vi "Time profile graph.vi"(8 "Assigned Time Profile plus":T1, 10 "time":dbl[](array[numeric]), 11 "Relative Data Array":dbl[](array[numeric])) -> (3 "Signal Time Graph":cluster{"time":dbl[], "current":dbl[]}[](graph))   [LabVIEW 2018]
panel:
  in  "Assigned Time Profile":T2
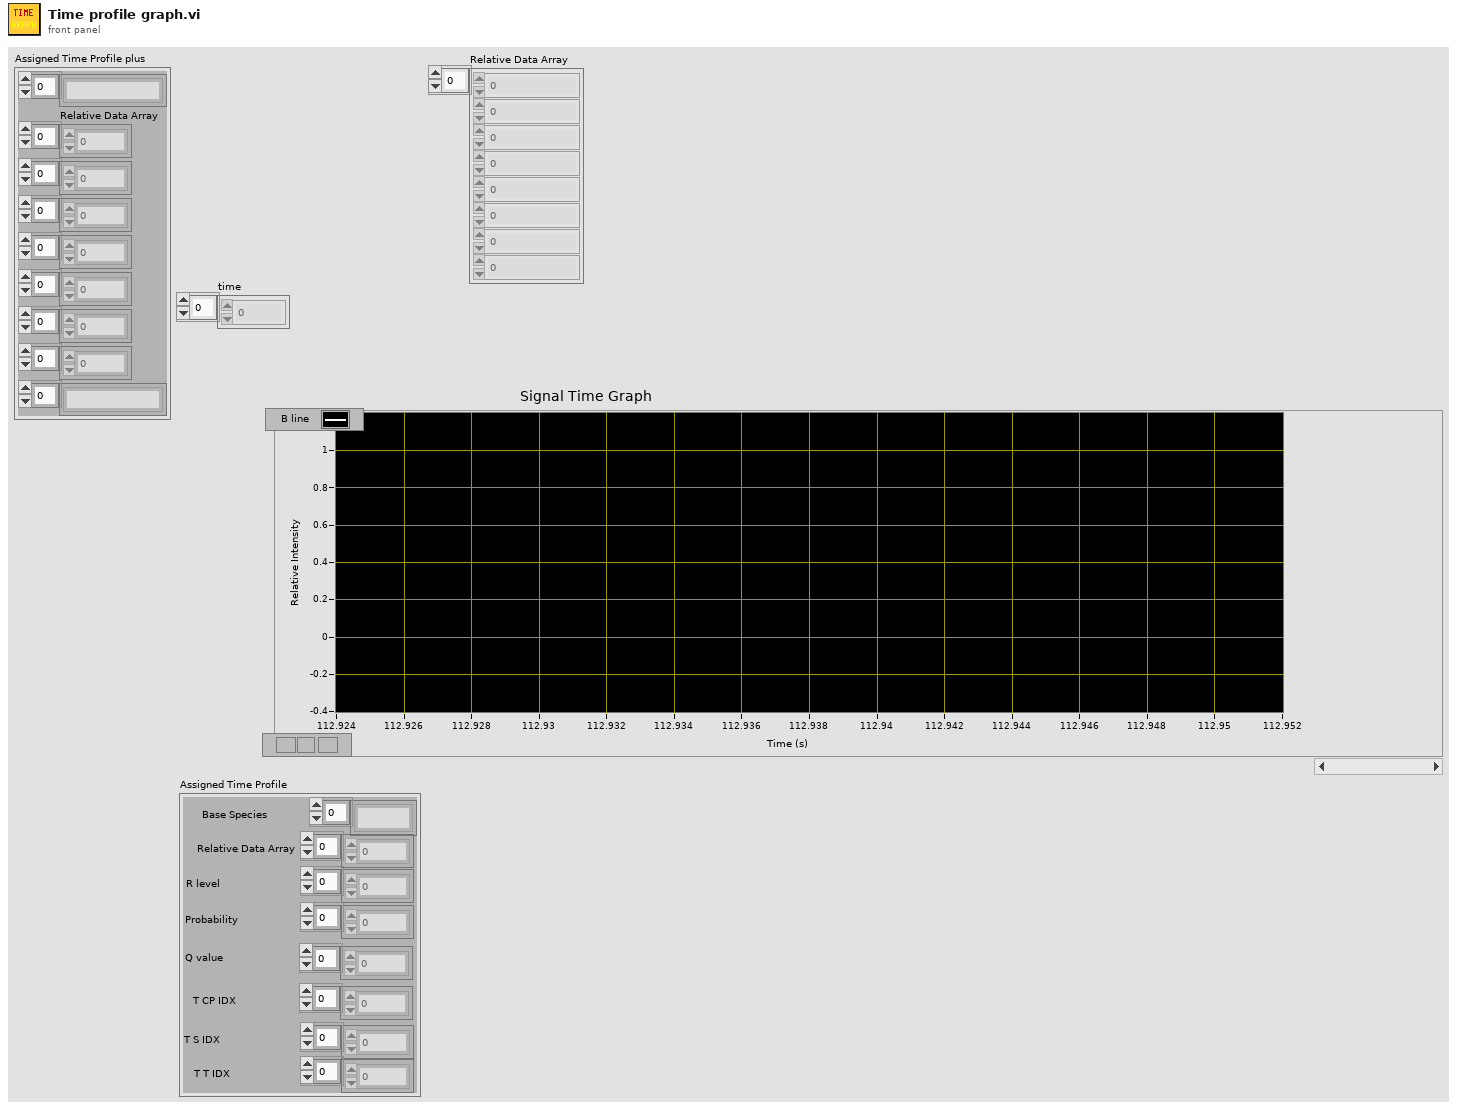
[diagram p1: front panel]
types:
  T1 = cluster{string[], "Relative Data Array":dbl[], dbl[], dbl[], dbl[], i32[], i32[], i32[], string[]}
  T2 = cluster{"Base Species":string[], "Relative Data Array":dbl[], "R level":dbl[], "Probability":dbl[], "Q value":dbl[], "T CP IDX":i32[], "T S IDX":i32[], "T T IDX":i32[]}
  T3 = cluster{"time":dbl[], "Relative Data Array":dbl[]}
  T4 = cluster{"time":dbl[], "Relative Data Array":dbl[]}[]
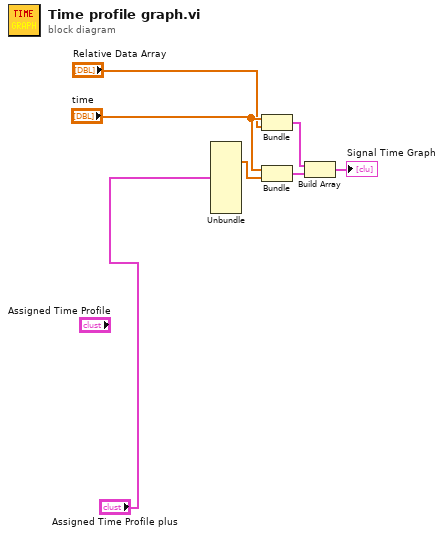
[diagram p0: block diagram]
diagram:
  n1 = Unbundle("Assigned Time Profile plus") -> (w2:dbl[])  [unwired: 8 out]
  n2 = Bundle("time"="time", "Relative Data Array"="Relative Data Array") -> (w7:T3)  [unwired: 1 in]
  n3 = Bundle("time"="time", w2) -> (w4:cluster{"time":dbl[], dbl[]})  [unwired: 1 in]
  n4 = Build Array(w7, w4) -> (→"Signal Time Graph":T4)
